vi "GPS_SUBVI.vi"(0 "String":string) -> (1 "LATITUD":dbl, 2 "LONGITUD":dbl)   [LabVIEW 2019]
panel:
  out "FIX":string
  out "Lon_R":string
  out "LONGITUD_S":string
  out "LAT_R":string
  out "LATITUD_S":string
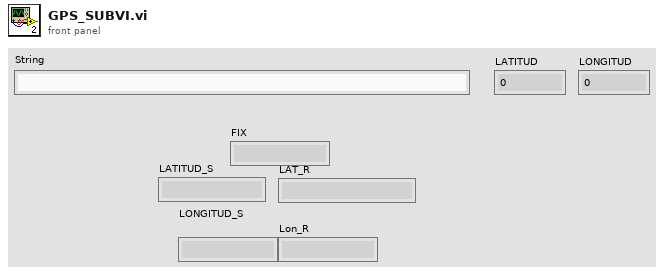
[diagram p1: front panel]
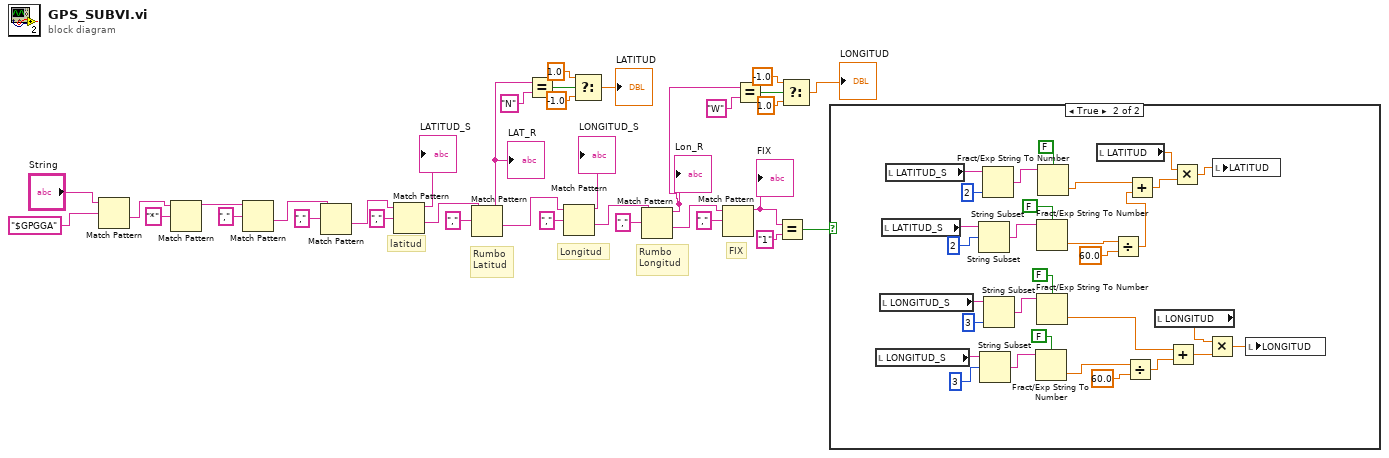
[diagram p0: block diagram]
diagram:
  # "FIX"
  # "Rumbo\nLongitud"
  # "Longitud"
  # "Rumbo\nLatitud"
  # "latitud"
  n1 = Match Pattern(string="String", regular expression="$GPGGA") -> (after substring=w32:string)  [unwired: 1 in, 3 out]
  n2 = Match Pattern(string=w32, regular expression="*") -> (before substring=w31:string)  [unwired: 1 in, 3 out]
  n3 = Match Pattern(string=w31, regular expression=",") -> (after substring=w28:string)  [unwired: 1 in, 3 out]
  n4 = Match Pattern(string=w28, regular expression=",") -> (after substring=w24:string)  [unwired: 1 in, 3 out]
  n5 = Match Pattern(string=w24, regular expression=",") -> (before substring=→"LATITUD_S":string, after substring=w25:string)  [unwired: 1 in, 2 out]
  n6 = Match Pattern(string=w25, regular expression=",") -> (before substring=w11:string, after substring=w20:string)  [unwired: 1 in, 2 out]
  "LAT_R" <- w11
  n7 = Equal?(x=w11, y="N") -> (x = y?=w12:bool)
  n8 = Match Pattern(string=w20, regular expression=",") -> (before substring=→"LONGITUD_S":string, after substring=w23:string)  [unwired: 1 in, 2 out]
  n9 = Select(t=1.0, s=w12, f=-1.0) -> (s? t:f=→"LATITUD":dbl)
  n10 = Match Pattern(string=w23, regular expression=",") -> (before substring=w2:string, after substring=w16:string)  [unwired: 1 in, 2 out]
  "Lon_R" <- w2
  n11 = Match Pattern(string=w16, regular expression=",") -> (before substring=w15:string)  [unwired: 1 in, 3 out]
  "FIX" <- w15
  n12 = Equal?(x=w2, y="W") -> (x = y?=w3:bool)
  n13 = Equal?(x=w15, y="1") -> (x = y?=w13:bool)
  n14 = Select(t=-1.0, s=w3, f=1.0) -> (s? t:f=→"LONGITUD":dbl)
  n15 = case shown="True" w13 {
    frame False {
    }
    frame True {
      n16 = local read "LONGITUD_S"() -> (w60:string)
      n17 = local read "LONGITUD_S"() -> (w58:string)
      n18 = local read "LATITUD_S"() -> (w63:string)
      n19 = local read "LATITUD_S"() -> (w65:string)
      n20 = String Subset(string=w63, offset (0)=2) -> (substring=w56:string)  [unwired: 1 in]
      n21 = String Subset(string=w60, offset (0)=3) -> (substring=w55:string)  [unwired: 1 in]
      n22 = String Subset(string=w65, length (rest)=2 ("length (rest)")) -> (substring=w57:string)  [unwired: 1 in]
      n23 = String Subset(string=w58, length (rest)=3 ("length (rest)")) -> (substring=w54:string)  [unwired: 1 in]
      n24 = Fract/Exp String To Number(use system decimal point (T)=FALSE, string=w55) -> (number=w46:dbl)  [unwired: 2 in, 1 out]
      n25 = Fract/Exp String To Number(use system decimal point (T)=FALSE, string=w56) -> (number=w49:dbl)  [unwired: 2 in, 1 out]
      n26 = Fract/Exp String To Number(use system decimal point (T)=FALSE, string=w54) -> (number=w42:dbl)  [unwired: 2 in, 1 out]
      n27 = Fract/Exp String To Number(use system decimal point (T)=FALSE, string=w57) -> (number=w45:dbl)  [unwired: 2 in, 1 out]
      n28 = local read "LATITUD"() -> (w38:dbl)
      n29 = Divide(x=w49, y=60.0) -> (x/y=w44:dbl)
      n30 = Divide(x=w46, y=60.0) -> (x/y=w43:dbl)
      n31 = Add(x=w45, y=w44) -> (x+y=w41:dbl)
      n32 = local read "LONGITUD"() -> (w37:dbl)
      n33 = Add(x=w42, y=w43) -> (x+y=w40:dbl)
      n34 = Multiply(x=w38, y=w41) -> (x*y=w39:dbl)
      n35 = Multiply(x=w37, y=w40) -> (x*y=w36:dbl)
      n36 = local write "LATITUD"(w39) -> ()
      n37 = local write "LONGITUD"(w36) -> ()
    }
  }
